vi "ConfigureLinkButton.vi"(6 "separator position left":i32, 7 "Separator":refnum<vi>, 8 "Position:Left":i32, 9 "is section header?":bool, 10 "GettingStartedWindow.lvlib:ClickableText.lvclass":refnum<class "ClickableText.lvclass">, 11 "Link Button 1":refnum<vi>) -> (0 "description":string, 1 "localized name":string, 2 "Top":i32, 3 "Link Button 2":refnum<vi>)   [LabVIEW 2023, in "GettingStartedWindow.lvlib"]
uses:
  <resource>/modes/FRC/GSW/GettingStartedWindow.lvlib
  <resource>/modes/FRC/GSW/Classes/ClickableText/ClickableText.lvclass
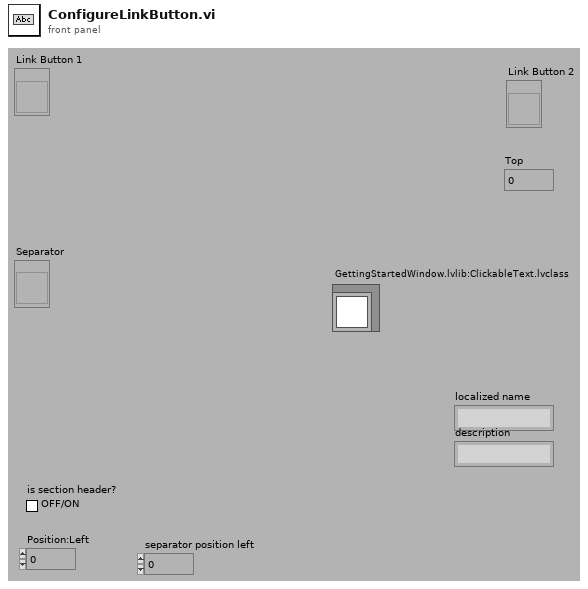
[diagram p1: front panel]
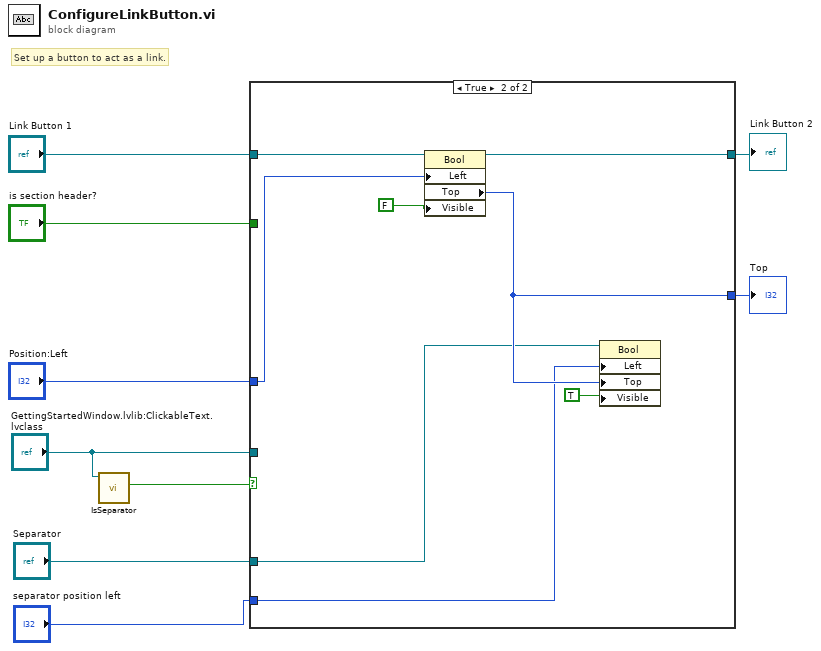
[diagram p0: block diagram]
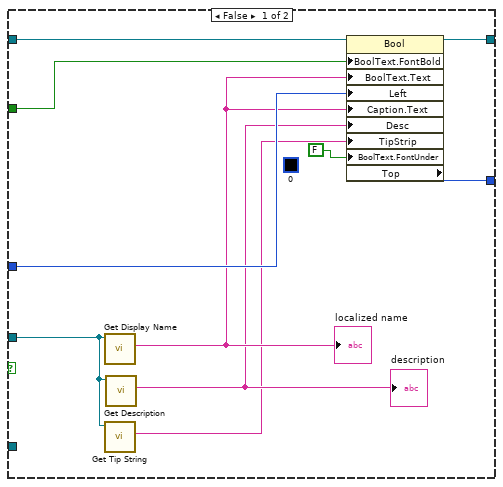
[diagram p2: hidden frame]
diagram:
  # "Set up a button to act as a link."
  n1 = call-dynamic "IsSeparator.vi"("Link in"="GettingStartedWindow.lvlib:ClickableText.lvclass") -> ("separator?"=w3:bool)  [unwired: 1 in, 9 out]
  n2 = case shown="True" w3 {
    tunnel: "Link Button 1" -> [w19 w27]
    tunnel: [w18 w23] -> w8
    tunnel: "is section header?" -> [w17 _]
    tunnel: "Position:Left" -> [w16 w26]
    tunnel: [w15 w24] -> w5
    tunnel: "GettingStartedWindow.lvlib:ClickableText.lvclass" -> [w10 _]
    tunnel: "Separator" -> [_ w22]
    tunnel: "separator position left" -> [_ w21]
    frame False {
      (unwired) u32 0
      n3 = call-dynamic "Get Display Name.vi"("ClickableText in"=w10) -> ("localized name"=w13:string)  [unwired: 1 in, 9 out]
      "localized name" <- w13
      n4 = call <resource>:"Get Tip String.vi"("ClickableText in"=w10) -> ("tip string"=w11:string)  [unwired: 1 in, 9 out]
      n5 = call <resource>:"Get Description.vi"("ClickableText in"=w10) -> ("description"=w12:string)  [unwired: 1 in, 9 out]
      "description" <- w12
      n6 = property class="Bool"(reference=w19, "BoolText.FontBold"=w17, "BoolText.Text"=w13, "Left"=w16, "Caption.Text"=w13, "Desc"=w12, "TipStrip"=w11, "BoolText.FontUnder"=FALSE ("Boolean Text.Font:Underline")) -> (reference out=w18:refnum<vi>, "Top"=w15:i32)  [unwired: 1 in, 1 out]
    }
    frame True {
      n7 = property class="Bool"(reference=w27, "Left"=w26, "Visible"=FALSE) -> (reference out=w23:refnum<vi>, "Top"=w24:i32)  [unwired: 1 in, 1 out]
      n8 = property class="Bool"(reference=w22, "Left"=w21, "Top"=w24, "Visible"=TRUE) -> ()  [unwired: 1 in, 2 out]
    }
  }
  "Link Button 2" <- w8
  "Top" <- w5
